vi "Exp - exec function error.vi"(5 "CE InstanceRef":T1, 6 "func name":string, 8 "CE error in":bool, 9 "error in":errorcluster) -> (2 "CE error out":bool)   [LabVIEW 2021]
doc: "::: CalcExpress Toolkit :::\nCopyright (c) 2000-2026 Konstantin Shifershteyn. All rights reserved."
uses:
  cetypes.llb/CalcExpress Instance RefNum.ctl
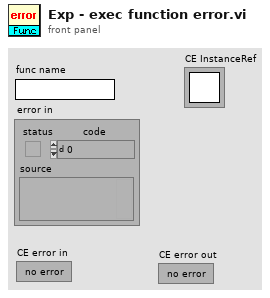
[diagram p1: front panel]
types:
  T1 = typedef "CalcExpress Instance RefNum.ctl" = refnum<k1>
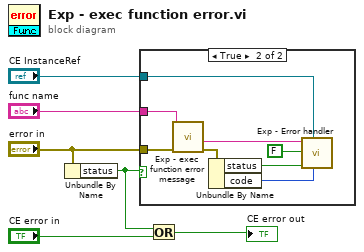
[diagram p0: block diagram]
diagram:
  n1 = Unbundle By Name("error in") -> ("status"=w2:bool)
  n2 = case shown="True" w2 {
    tunnel: "error in" -> [_ w13]
    tunnel: "func name" -> [_ w12]
    tunnel: "CE InstanceRef" -> [_ w7]
    frame False {
    }
    frame True {
      n3 = call "Exp - exec function error message.vi"("error in"=w13, "func name"=w12) -> ("error out"=w9:errorcluster, "error message"=w11:string)  [unwired: 6 in]
      n4 = Unbundle By Name(w9) -> ("status"=w10:bool, "code"=w8:i32)
      n5 = call "Exp - Error handler.vi"("error code in"=w8, "InstanceRef"=w7, "error in"=w10, "add FuncName (T)"=FALSE, "error message in"=w11) -> ()  [unwired: 4 in, 3 out]
    }
  }
  n6 = Or(x=w2, y="CE error in") -> (x .or. y?=→"CE error out":bool)
